vi "VIH ProjFile - Group Rule - Convert Paths.vi"(7 "Root Dir":path, 9 "Master Rule (F)":bool, 10 "Operation":enum16{"Read", "Write"}(ring), 11 "Group Rule":T1) -> (3 "Group Rule out":T1)   [LabVIEW 2014]
doc: "::: VI Helpeks :::\nCopyright (c) 2000-2026 Konstantin Shifershteyn. All rights reserved."
uses:
  _VIH HelpGen.llb/VIH HelpGen Typedef - Cluster - Group Rule.ctl
  _VIH HelpGen.llb/VIH HelpGen Typedef - Enum - Default,Enable,Disable.ctl
  _VIH HelpGen.llb/VIH HelpGen Typedef - Cluster - Group Rule - Source Paths.ctl
  _VIH HelpGen.llb/VIH HelpGen Typedef - Cluster - Group Rule - Target Paths.ctl
  _VIH HelpGen.llb/VIH HelpGen Typedef - Enum - Description Mode.ctl
  _VIH HelpGen.llb/VIH HelpGen Typedef - Cluster - Control Rule.ctl
  _VIH HelpGen.llb/VIH HelpGen Typedef - Cluster - Enum Value Info.ctl
  _VIH HelpGen.llb/VIH HelpGen Typedef - Cluster - Group Rule - Flags.ctl
panel:
  # "VI Helpeks\nCopyright (c) 2012-2026 Konstantin Shifershteyn"
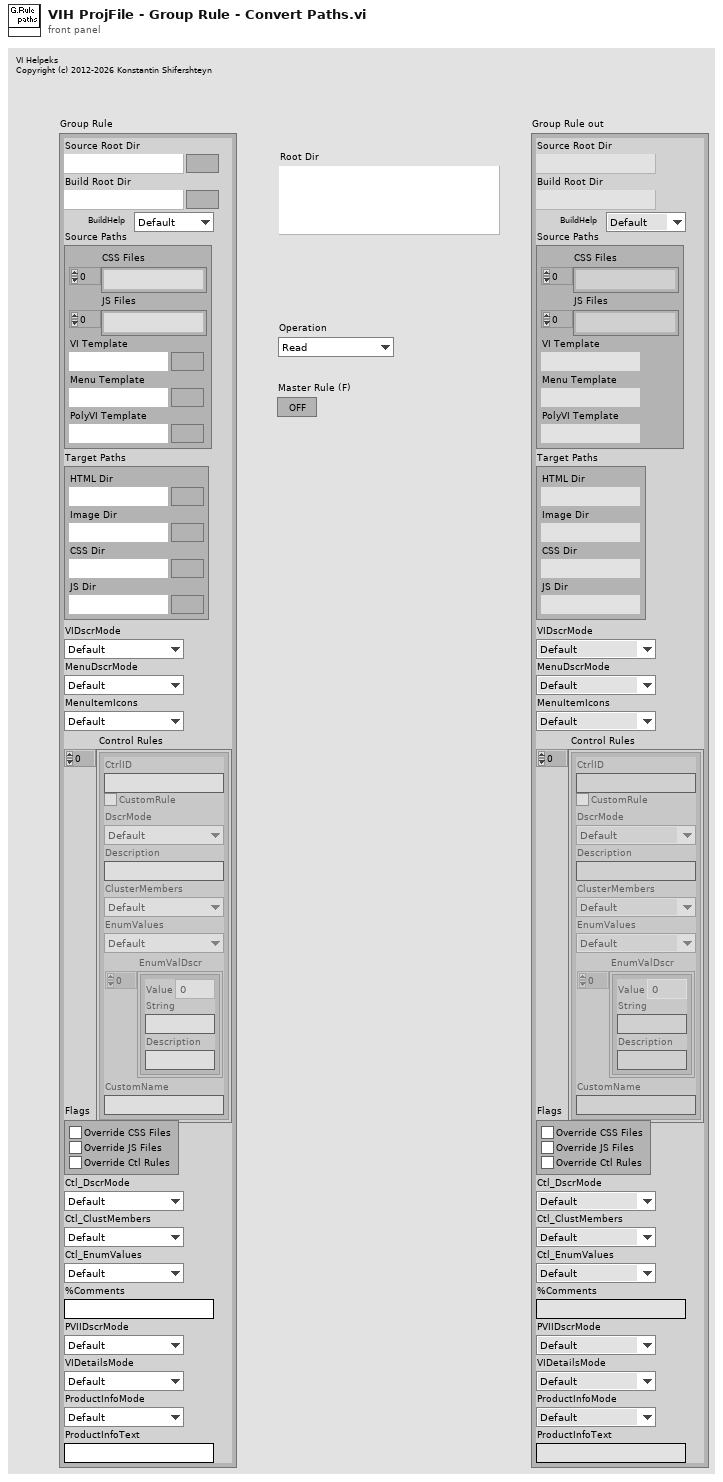
[diagram p1: front panel]
types:
  T1 = typedef "VIH HelpGen Typedef - Cluster - Group Rule.ctl" = cluster{"Source Root Dir":path, "Build Root Dir":path, "BuildHelp":T2, "Source Paths":T3, "Target Paths":T4, "VIDscrMode":T5, "MenuDscrMode":T5, "MenuItemIcons":T2, "Control Rules":T6[], "Flags":T8, "Ctl_DscrMode":T5, "Ctl_ClustMembers":T2, "Ctl_EnumValues":T2, "%Comments":string, "PVIIDscrMode":T5, "VIDetailsMode":T5, "ProductInfoMode":T2, "ProductInfoText":string}
  T2 = typedef "VIH HelpGen Typedef - Enum - Default,Enable,Disable.ctl" = enum16{"Default", "Enable", "Disable"}
  T3 = typedef "VIH HelpGen Typedef - Cluster - Group Rule - Source Paths.ctl" = cluster{"CSS Files":path[], "JS Files":path[], "VI Template":path, "Menu Template":path, "PolyVI Template":path}
  T4 = typedef "VIH HelpGen Typedef - Cluster - Group Rule - Target Paths.ctl" = cluster{"HTML Dir":path, "Image Dir":path, "CSS Dir":path, "JS Dir":path}
  T5 = typedef "VIH HelpGen Typedef - Enum - Description Mode.ctl" = enum16{"Default", "Description", "Description1", "Description2", "Custom", "None"}
  T6 = typedef "VIH HelpGen Typedef - Cluster - Control Rule.ctl" = cluster{"CtrlID":string, "CustomRule":bool, "DscrMode":T5, "Description":string, "ClusterMembers":T2, "EnumValues":T2, "EnumValDscr":T7[], "CustomName":string}
  T7 = typedef "VIH HelpGen Typedef - Cluster - Enum Value Info.ctl" = cluster{"Value":ext, "String":string, "Description":string}
  T8 = typedef "VIH HelpGen Typedef - Cluster - Group Rule - Flags.ctl" = cluster{"Override CSS Files":bool, "Override JS Files":bool, "Override Ctl Rules":bool}
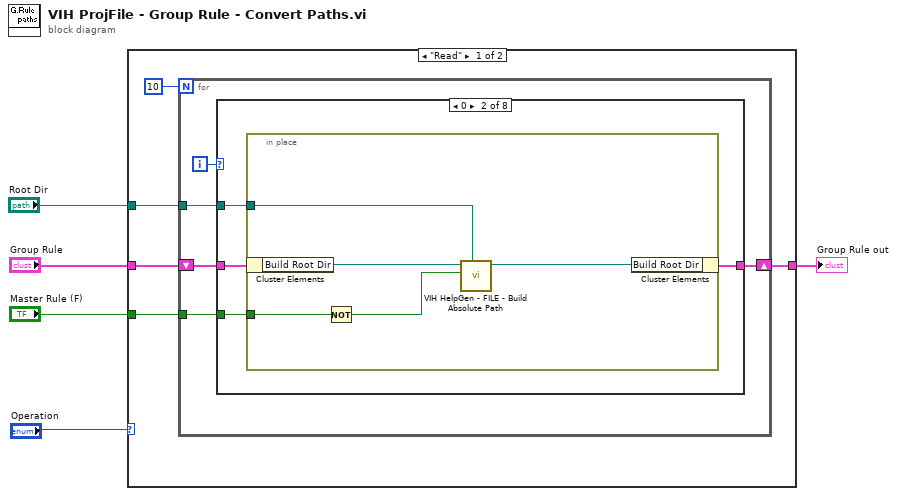
[diagram p0: block diagram]
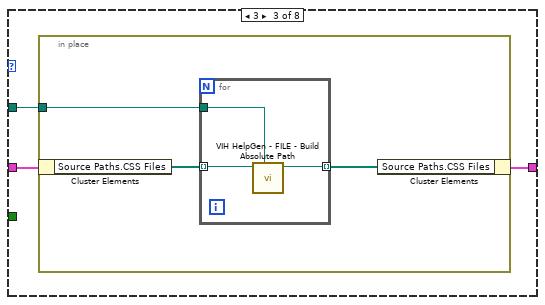
[diagram p3: hidden frame]
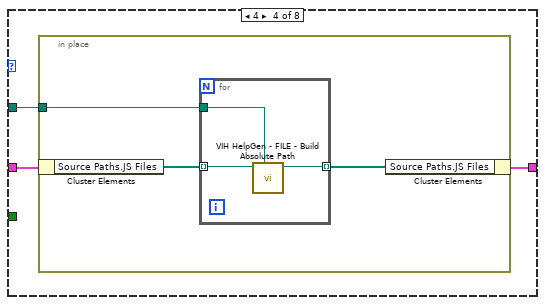
[diagram p4: hidden frame]
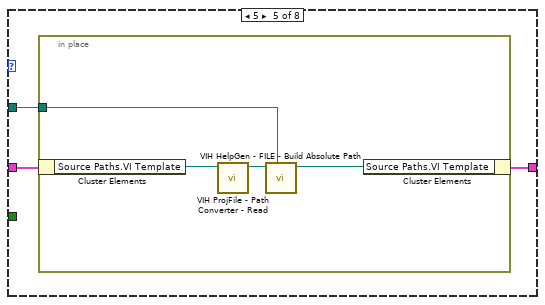
[diagram p5: hidden frame]
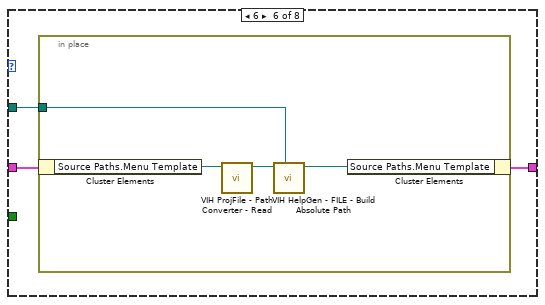
[diagram p6: hidden frame]
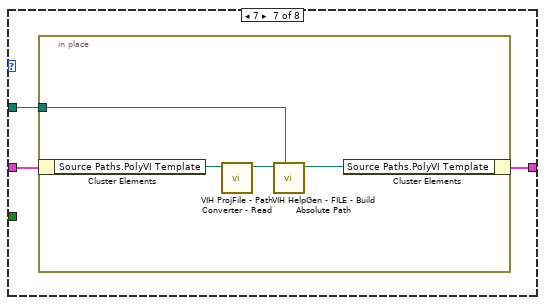
[diagram p7: hidden frame]
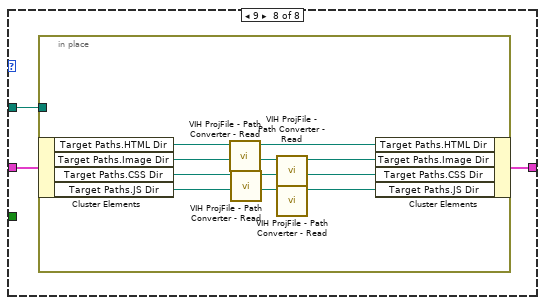
[diagram p8: hidden frame]
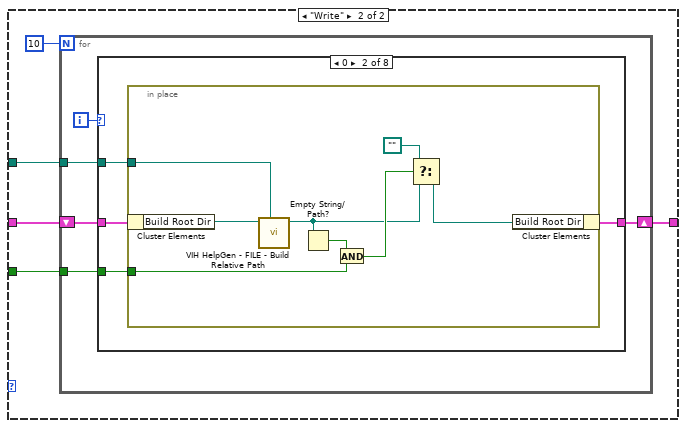
[diagram p9: hidden frame]
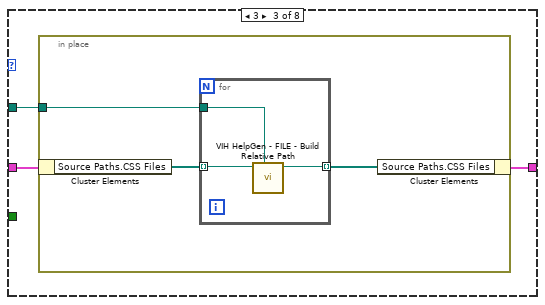
[diagram p11: hidden frame]
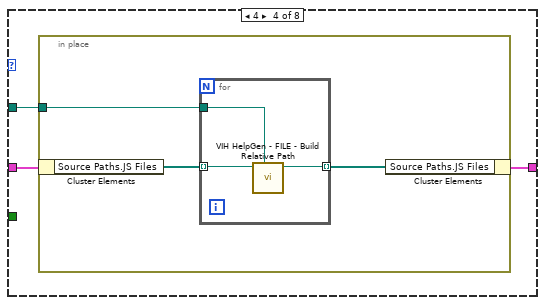
[diagram p12: hidden frame]
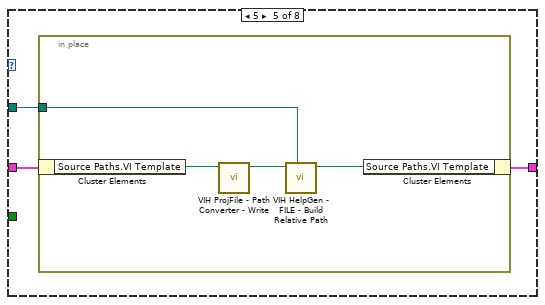
[diagram p13: hidden frame]
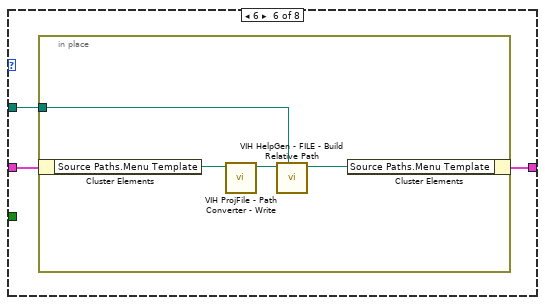
[diagram p14: hidden frame]
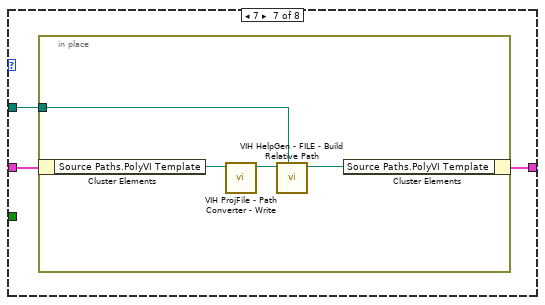
[diagram p15: hidden frame]
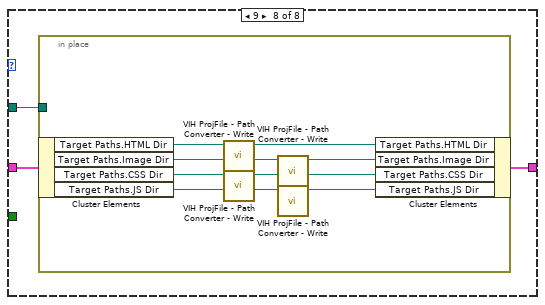
[diagram p16: hidden frame]
diagram:
  n1 = case shown="\"Read\"" "Operation" {
    tunnel: "Group Rule" -> [w10 w80]
    tunnel: [w9 w79] -> w4
    tunnel: "Root Dir" -> [w7 w77]
    tunnel: "Master Rule (F)" -> [w6 w76]
    frame "Read" {
      n2 = for {
        N: 10 -> [_]
        shift-right: [w14] -> w9
        shift-left: w10 -> [w13]
        tunnel: w7 -> [w12]
        tunnel: w6 -> [w11]
        i -> [w15]
        n3 = case shown="0" w15 {
          tunnel: [w16 w19 w27 w36 w45 w52 w59 w66] -> w14
          tunnel: w13 -> [w16 w20 w28 w37 w46 w53 w60 w67]
          tunnel: w12 -> [_ w18 w26 w35 w44 w51 w58 w65]
          tunnel: w11 -> [_ w17 _ _ _ _ _ _]
          frame Default {
          }
          frame 0 {
            n4 = in-place {
              in-place-border: w18 -> [w24]
              in-place-border: w17 -> [w22]
              n5 = in-place-cluster #1(w20) -> ("Build Root Dir"=w25:path)
              n6 = Not(x=w22) -> (.not. x?=w21:bool)
              n7 = call "VIH HelpGen - FILE - Build Absolute Path.vi"("Root Path"=w24, "Allow Empty Path (T)"=w21, "Path in"=w25) -> ("Path out"=w23:path)  [unwired: 8 in]
              n8 = in-place-cluster #1("Build Root Dir"=w23) -> (w19:T1)
            }
          }
          frame 3 {
            n9 = in-place {
              in-place-border: w26 -> [w30]
              n10 = in-place-cluster #2(w28) -> ("Source Paths.CSS Files"=w31:path[])
              n11 = for {
                tunnel: w31 -> [w34] mode=indexing
                tunnel: w30 -> [w33]
                tunnel: [w32] -> w29 mode=indexing
                n12 = call "VIH HelpGen - FILE - Build Absolute Path.vi"("Root Path"=w33, "Path in"=w34) -> ("Path out"=w32:path)  [unwired: 9 in]
              }
              n13 = in-place-cluster #2("Source Paths.CSS Files"=w29) -> (w27:T1)
            }
          }
          frame 4 {
            n14 = in-place {
              in-place-border: w35 -> [w39]
              n15 = in-place-cluster #3(w37) -> ("Source Paths.JS Files"=w40:path[])
              n16 = for {
                tunnel: w40 -> [w43] mode=indexing
                tunnel: w39 -> [w42]
                tunnel: [w41] -> w38 mode=indexing
                n17 = call "VIH HelpGen - FILE - Build Absolute Path.vi"("Root Path"=w42, "Path in"=w43) -> ("Path out"=w41:path)  [unwired: 9 in]
              }
              n18 = in-place-cluster #3("Source Paths.JS Files"=w38) -> (w36:T1)
            }
          }
          frame 5 {
            n19 = in-place {
              in-place-border: w44 -> [w50]
              n20 = in-place-cluster #4(w46) -> ("Source Paths.VI Template"=w48:path)
              n21 = call "VIH ProjFile - Path Converter - Read.vi"("Path in"=w48) -> ("Path out"=w47:path)  [unwired: 10 in]
              n22 = call "VIH HelpGen - FILE - Build Absolute Path.vi"("Root Path"=w50, "Path in"=w47) -> ("Path out"=w49:path)  [unwired: 9 in]
              n23 = in-place-cluster #4("Source Paths.VI Template"=w49) -> (w45:T1)
            }
          }
          frame 6 {
            n24 = in-place {
              in-place-border: w51 -> [w57]
              n25 = in-place-cluster #5(w53) -> ("Source Paths.Menu Template"=w55:path)
              n26 = call "VIH ProjFile - Path Converter - Read.vi"("Path in"=w55) -> ("Path out"=w54:path)  [unwired: 10 in]
              n27 = call "VIH HelpGen - FILE - Build Absolute Path.vi"("Root Path"=w57, "Path in"=w54) -> ("Path out"=w56:path)  [unwired: 9 in]
              n28 = in-place-cluster #5("Source Paths.Menu Template"=w56) -> (w52:T1)
            }
          }
          frame 7 {
            n29 = in-place {
              in-place-border: w58 -> [w64]
              n30 = in-place-cluster #6(w60) -> ("Source Paths.PolyVI Template"=w62:path)
              n31 = call "VIH ProjFile - Path Converter - Read.vi"("Path in"=w62) -> ("Path out"=w61:path)  [unwired: 10 in]
              n32 = call "VIH HelpGen - FILE - Build Absolute Path.vi"("Root Path"=w64, "Path in"=w61) -> ("Path out"=w63:path)  [unwired: 9 in]
              n33 = in-place-cluster #6("Source Paths.PolyVI Template"=w63) -> (w59:T1)
            }
          }
          frame 9 {
            n34 = in-place {
              in-place-border: w65 -> [_]
              n35 = in-place-cluster #7(w67) -> ("Target Paths.HTML Dir"=w75:path, "Target Paths.Image Dir"=w73:path, "Target Paths.CSS Dir"=w71:path, "Target Paths.JS Dir"=w69:path)
              n36 = call "VIH ProjFile - Path Converter - Read.vi"("Path in"=w75) -> ("Path out"=w74:path)  [unwired: 10 in]
              n37 = call "VIH ProjFile - Path Converter - Read.vi"("Path in"=w71) -> ("Path out"=w70:path)  [unwired: 10 in]
              n38 = call "VIH ProjFile - Path Converter - Read.vi"("Path in"=w73) -> ("Path out"=w72:path)  [unwired: 10 in]
              n39 = call "VIH ProjFile - Path Converter - Read.vi"("Path in"=w69) -> ("Path out"=w68:path)  [unwired: 10 in]
              n40 = in-place-cluster #7("Target Paths.HTML Dir"=w74, "Target Paths.Image Dir"=w72, "Target Paths.CSS Dir"=w70, "Target Paths.JS Dir"=w68) -> (w66:T1)
            }
          }
        }
      }
    }
    frame "Write" {
      n41 = for {
        N: 10 -> [_]
        shift-right: [w84] -> w79
        shift-left: w80 -> [w83]
        tunnel: w77 -> [w82]
        tunnel: w76 -> [w81]
        i -> [w85]
        n42 = case shown="0" w85 {
          tunnel: [w86 w89 w100 w109 w118 w125 w132 w139] -> w84
          tunnel: w83 -> [w86 w90 w101 w110 w119 w126 w133 w140]
          tunnel: w82 -> [_ w88 w99 w108 w117 w124 w131 w138]
          tunnel: w81 -> [_ w87 _ _ _ _ _ _]
          frame Default {
          }
          frame 0 {
            n43 = in-place {
              in-place-border: w88 -> [w97]
              in-place-border: w87 -> [w91]
              n44 = in-place-cluster #8(w90) -> ("Build Root Dir"=w98:path)
              n45 = call "VIH HelpGen - FILE - Build Relative Path.vi"("Root Path"=w97, "Path in"=w98) -> ("Path out"=w95:path)  [unwired: 9 in]
              n46 = Empty String/Path?(string/path=w95) -> (empty?=w92:bool)
              n47 = And(x=w92, y=w91) -> (x .and. y?=w96:bool)
              n48 = Select(t=path "", s=w96, f=w95) -> (s? t:f=w94:path)
              n49 = in-place-cluster #8("Build Root Dir"=w94) -> (w89:T1)
            }
          }
          frame 3 {
            n50 = in-place {
              in-place-border: w99 -> [w103]
              n51 = in-place-cluster #9(w101) -> ("Source Paths.CSS Files"=w104:path[])
              n52 = for {
                tunnel: w104 -> [w107] mode=indexing
                tunnel: w103 -> [w106]
                tunnel: [w105] -> w102 mode=indexing
                n53 = call "VIH HelpGen - FILE - Build Relative Path.vi"("Root Path"=w106, "Path in"=w107) -> ("Path out"=w105:path)  [unwired: 9 in]
              }
              n54 = in-place-cluster #9("Source Paths.CSS Files"=w102) -> (w100:T1)
            }
          }
          frame 4 {
            n55 = in-place {
              in-place-border: w108 -> [w112]
              n56 = in-place-cluster #10(w110) -> ("Source Paths.JS Files"=w113:path[])
              n57 = for {
                tunnel: w113 -> [w116] mode=indexing
                tunnel: w112 -> [w115]
                tunnel: [w114] -> w111 mode=indexing
                n58 = call "VIH HelpGen - FILE - Build Relative Path.vi"("Root Path"=w115, "Path in"=w116) -> ("Path out"=w114:path)  [unwired: 9 in]
              }
              n59 = in-place-cluster #10("Source Paths.JS Files"=w111) -> (w109:T1)
            }
          }
          frame 5 {
            n60 = in-place {
              in-place-border: w117 -> [w123]
              n61 = in-place-cluster #11(w119) -> ("Source Paths.VI Template"=w121:path)
              n62 = call "VIH ProjFile - Path Converter - Write.vi"("Path in"=w121) -> ("Path out"=w120:path)  [unwired: 10 in]
              n63 = call "VIH HelpGen - FILE - Build Relative Path.vi"("Root Path"=w123, "Path in"=w120) -> ("Path out"=w122:path)  [unwired: 9 in]
              n64 = in-place-cluster #11("Source Paths.VI Template"=w122) -> (w118:T1)
            }
          }
          frame 6 {
            n65 = in-place {
              in-place-border: w124 -> [w130]
              n66 = in-place-cluster #12(w126) -> ("Source Paths.Menu Template"=w128:path)
              n67 = call "VIH ProjFile - Path Converter - Write.vi"("Path in"=w128) -> ("Path out"=w127:path)  [unwired: 10 in]
              n68 = call "VIH HelpGen - FILE - Build Relative Path.vi"("Root Path"=w130, "Path in"=w127) -> ("Path out"=w129:path)  [unwired: 9 in]
              n69 = in-place-cluster #12("Source Paths.Menu Template"=w129) -> (w125:T1)
            }
          }
          frame 7 {
            n70 = in-place {
              in-place-border: w131 -> [w137]
              n71 = in-place-cluster #13(w133) -> ("Source Paths.PolyVI Template"=w135:path)
              n72 = call "VIH ProjFile - Path Converter - Write.vi"("Path in"=w135) -> ("Path out"=w134:path)  [unwired: 10 in]
              n73 = call "VIH HelpGen - FILE - Build Relative Path.vi"("Root Path"=w137, "Path in"=w134) -> ("Path out"=w136:path)  [unwired: 9 in]
              n74 = in-place-cluster #13("Source Paths.PolyVI Template"=w136) -> (w132:T1)
            }
          }
          frame 9 {
            n75 = in-place {
              in-place-border: w138 -> [_]
              n76 = in-place-cluster #14(w140) -> ("Target Paths.HTML Dir"=w148:path, "Target Paths.Image Dir"=w146:path, "Target Paths.CSS Dir"=w144:path, "Target Paths.JS Dir"=w142:path)
              n77 = call "VIH ProjFile - Path Converter - Write.vi"("Path in"=w148) -> ("Path out"=w147:path)  [unwired: 10 in]
              n78 = call "VIH ProjFile - Path Converter - Write.vi"("Path in"=w144) -> ("Path out"=w143:path)  [unwired: 10 in]
              n79 = call "VIH ProjFile - Path Converter - Write.vi"("Path in"=w146) -> ("Path out"=w145:path)  [unwired: 10 in]
              n80 = call "VIH ProjFile - Path Converter - Write.vi"("Path in"=w142) -> ("Path out"=w141:path)  [unwired: 10 in]
              n81 = in-place-cluster #14("Target Paths.HTML Dir"=w147, "Target Paths.Image Dir"=w145, "Target Paths.CSS Dir"=w143, "Target Paths.JS Dir"=w141) -> (w139:T1)
            }
          }
        }
      }
    }
  }
  "Group Rule out" <- w4
